vi "test tools list error descriptions.vi"(8 "error in (no error)":errorcluster) -> (0 "error out":errorcluster, 2 "tool entry":string, 3 "body":string)   [LabVIEW 2020, in "MCP Server tests.lvlib"]
doc: "tools/list leaves out LabVIEW's default error cluster descriptions. For fake_tool_error_descriptions, error in (no error) in inputSchema and error out in outputSchema carry the help text of NI's Error In 3D and Error Out 3D controls, elements included. In tools/list neither they nor their status, code and source elements have a description key, while their type is still there. The descriptions the tool's author wrote are kept unchanged: previous error (input) and its source element, last error (output) and its code element, and last error.status, whose NI text has a sentence added. Their other elements, which carry NI's defaults, have none - including previous error.code, whose default text has CR LF line breaks and white space around it. The request is sent with the LabVIEW HTTP Client directly."
uses:
  MCP Server tests.lvlib
  9d4e3eac-005d-49bf-aed6-dfa1cae0cf6b.vi
  <vilib>/JDP Science/JSONtext/Next JSON Value.vi
  <vilib>/JDP Science/JSONtext/String Subset.vi
  <vilib>/JDP Science/JSONtext/Parsing/Advance past next JSON Value (inlined COPY).vi
  <vilib>/JDP Science/JSONtext/Parsing/Advance past whitespace.vi
  <vilib>/JDP Science/JSONtext/Parsing/Advance past String.vi
  <vilib>/JDP Science/JSONtext/Parsing/Advance past Number.vi
  <vilib>/JDP Science/JSONtext/Parsing/Advance past Line Ending.vi
  <vilib>/JDP Science/JSONtext/Parsing/Parse Full Path or Item Name.vi
  <vilib>/JDP Science/JSONtext/Parsing/Advance past Array.vi
  <vilib>/JDP Science/JSONtext/Parsing/Advance past Object.vi
  <vilib>/JDP Science/JSONtext/support/Error Cluster From Code.vi
  <vilib>/JDP Science/JSONtext/Offset/Find Item Locations by Path.vi
  <vilib>/JDP Science/JSONtext/JSON text to Variant.vi
  <vilib>/JDP Science/JSONtext/LVClass Serializer/JSONtext LVClass Serializer.lvclass
  <vilib>/addons/_JKI Toolkits/Caraya/classes/Test/Test.lvclass
  <vilib>/JDP Science/JSONtext/JSONtext.lvlib
  <vilib>/addons/_JKI Toolkits/Caraya/classes/Assert/Assert.lvclass
panel:
  out "lookup error":errorcluster
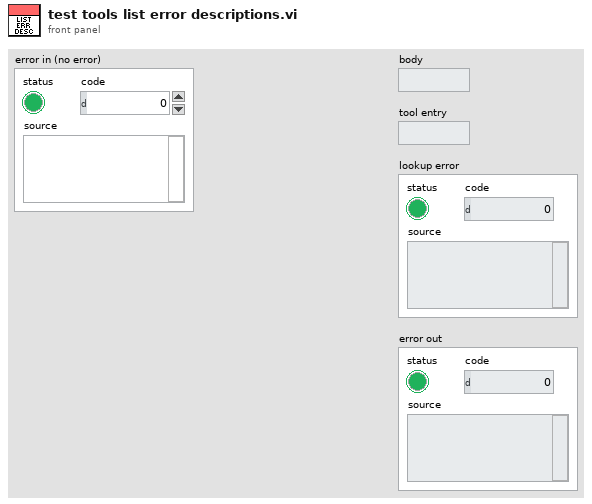
[diagram p1: front panel]
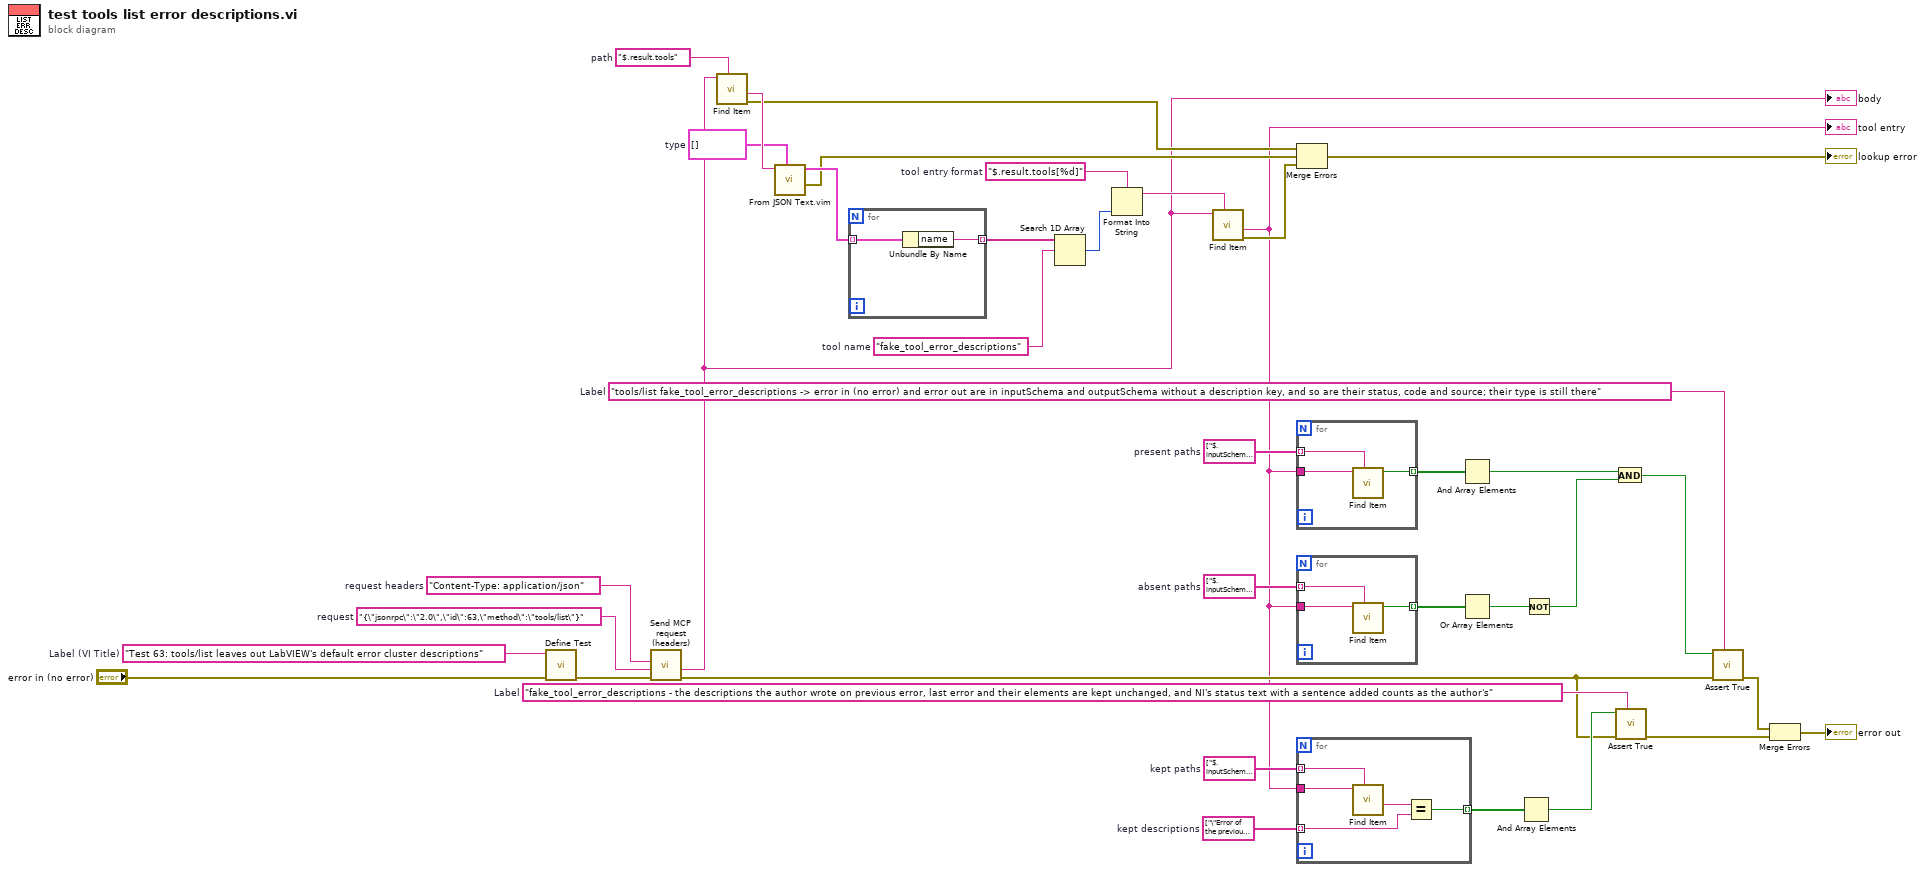
[diagram p0: block diagram]
diagram:
  w36 = "Content-Type: application/json"  # request headers
  w12 = "fake_tool_error_descriptions - the descriptions the author wrote on previous error, last error and their elements are kept unchanged, and NI's status text with a sentence added counts as the author's"  # Label
  w7 = "tools/list fake_tool_error_descriptions -> error in (no error) and error out are in inputSchema and outputSchema without a description key, and so are their status, code and source; their type is still there"  # Label
  w18 = string[] ["\"Error of the previous run of the tool.\"", "\"Where the previous error came from.\"", "\"The last error the device reported.\"", "\"Device error code.\""]  # kept descriptions
  w19 = string[] ["$.inputSchema.properties.previous_error.description", "$.inputSchema.properties.previous_error.properties.source.description", "$.outputSchema.properties.last_error.description", "$.outputSchema.properties.last_error.properties.code.description"]  # kept paths
  w20 = string[] ["$.inputSchema.properties.error_in__no_error_.description", "$.inputSchema.properties.error_in__no_error_.properties.status.description", "$.inputSchema.properties.error_in__no_error_.properties.code.description", "$.inputSchema.properties.error_in__no_error_.properties.source.description", "$.outputSchema.properties.error_out.description", "$.outputSchema.properties.error_out.properties.status.description", "$.outputSchema.properties.error_out.properties.code.description", "$.outputSchema.properties.error_out.properties.source.description", "$.inputSchema.properties.previous_error.properties.status.description", "$.inputSchema.properties.previous_error.properties.code.description", "$.outputSchema.properties.last_error.properties.source.description"]  # absent paths
  w21 = string[] ["$.inputSchema.properties.error_in__no_error_.type", "$.inputSchema.properties.error_in__no_error_.properties.status.type", "$.inputSchema.properties.error_in__no_error_.properties.code.type", "$.inputSchema.properties.error_in__no_error_.properties.source.type", "$.outputSchema.properties.error_out.type", "$.outputSchema.properties.error_out.properties.status.type", "$.outputSchema.properties.error_out.properties.code.type", "$.outputSchema.properties.error_out.properties.source.type", "$.outputSchema.properties.last_error.properties.status.description"]  # present paths
  w26 = "$.result.tools[%d]"  # tool entry format
  w28 = "fake_tool_error_descriptions"  # tool name
  w31 = cluster{"name":string}[] []  # type
  w33 = "$.result.tools"  # path
  w35 = "{\"jsonrpc\":\"2.0\",\"id\":63,\"method\":\"tools/list\"}"  # request
  w38 = "Test 63: tools/list leaves out LabVIEW's default error cluster descriptions"  # Label (VI Title)
  n1 = call <vilib>:"Define Test.vi"("error in (no error)"="error in (no error)", "Label (VI Title)"=w38) -> ("error out"=w34:errorcluster)  [unwired: 8 in, 1 out]
  n2 = call "Send MCP request (headers).vi"("error in (no error)"=w34, "request"=w35, "request headers"=w36) -> ("error out"=w8:errorcluster, "response"=w4:string)  [unwired: 5 in, 2 out]
  "body" <- w4
  n3 = call <vilib>:"Find Item.vi"("$Path or Item Name"=w33, "JSON"=w4) -> ("error out"=w24:errorcluster, "<JSON>"=w32:string)  [unwired: 6 in, 2 out]
  n4 = call "From JSON Text.vim"("Data Type and Default Value"=w31, "JSON"=w32) -> ("error out"=w23:errorcluster, "Data out"=w30:cluster{"name":string}[])  [unwired: 8 in]
  n5 = for {
    tunnel: w30 -> [w40] mode=indexing
    tunnel: [w39] -> w29 mode=indexing
    n6 = Unbundle By Name(w40) -> ("name"=w39:string)
  }
  n7 = Search 1D Array(1D array=w29, element=w28) -> (index of element=w27:i32)  [unwired: 1 in]
  n8 = Format Into String(format string=w26, w27) -> (resulting string=w25:string)  [unwired: 2 in, 1 out]
  n9 = call <vilib>:"Find Item.vi"("$Path or Item Name"=w25, "JSON"=w4) -> ("error out"=w22:errorcluster, "<JSON>"=w3:string)  [unwired: 6 in, 2 out]
  "tool entry" <- w3
  n10 = Merge Errors(w24, w23, w22) -> (→"lookup error":errorcluster)
  n11 = for {
    tunnel: w21 -> [w42] mode=indexing
    tunnel: w3 -> [w43]
    tunnel: [w41] -> w17 mode=indexing
    n12 = call <vilib>:"Find Item.vi"("$Path or Item Name"=w42, "JSON"=w43) -> ("Found"=w41:bool)  [unwired: 6 in, 3 out]
  }
  n13 = for {
    tunnel: w20 -> [w45] mode=indexing
    tunnel: w3 -> [w46]
    tunnel: [w44] -> w16 mode=indexing
    n14 = call <vilib>:"Find Item.vi"("$Path or Item Name"=w45, "JSON"=w46) -> ("Found"=w44:bool)  [unwired: 6 in, 3 out]
  }
  n15 = for {
    tunnel: w19 -> [w50] mode=indexing
    tunnel: w18 -> [w48] mode=indexing
    tunnel: w3 -> [w51]
    tunnel: [w47] -> w15 mode=indexing
    n16 = call <vilib>:"Find Item.vi"("$Path or Item Name"=w50, "JSON"=w51) -> ("<JSON>"=w49:string)  [unwired: 6 in, 3 out]
    n17 = Equal?(x=w49, y=w48) -> (x = y?=w47:bool)
  }
  n18 = And Array Elements(Boolean array=w17) -> (logical AND=w11:bool)
  n19 = Or Array Elements(Boolean array=w16) -> (logical OR=w14:bool)
  n20 = And Array Elements(Boolean array=w15) -> (logical AND=w13:bool)
  n21 = Not(x=w14) -> (.not. x?=w10:bool)
  n22 = And(x=w11, y=w10) -> (x .and. y?=w9:bool)
  n23 = call <vilib>:"Assert True.vi"("Label"=w12, "error in (no error)"=w8, "True?"=w13) -> ("error out"=w5:errorcluster)  [unwired: 7 in, 1 out]
  n24 = call <vilib>:"Assert True.vi"("Label"=w7, "error in (no error)"=w8, "True?"=w9) -> ("error out"=w6:errorcluster)  [unwired: 7 in, 1 out]
  n25 = Merge Errors(w6, w5) -> (→"error out":errorcluster)
